vi "Update.vi"(9 "log line":string, 10 "file ref":refnum<file>, 11 "size trigger in":refnum<class "RolloverTrigger.Size.lvclass">) -> (3 "size trigger out":refnum<class "RolloverTrigger.Size.lvclass">)   [LabVIEW 2018, in "GLog.lvlib" / "RolloverTrigger.Size.lvclass"]
doc: "Updates the current file size without touching the filesystem."
uses:
  RolloverTrigger.Size.lvclass
  RolloverTrigger.Size.lvclass/RolloverTrigger.Size.ctl
  d0e10f38-aaa8-410d-b386-210e52cdc805.vi
panel:
  # "Connector Pane"
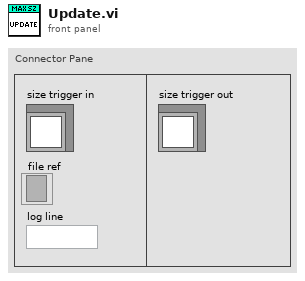
[diagram p1: front panel]
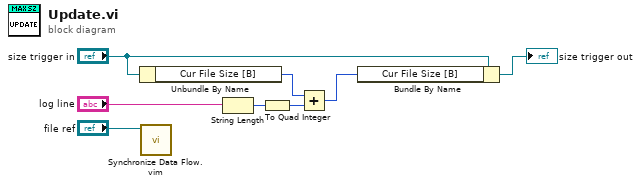
[diagram p0: block diagram]
diagram:
  n1 = Unbundle By Name("size trigger in") -> ("Cur File Size [B]"=w5:i64)
  n2 = call "Synchronize Data Flow.vim"("input 1"="file ref") -> ()  [unwired: 3 in, 4 out]
  n3 = String Length(string="log line") -> (length=w4:i32)
  n4 = To Quad Integer(1:w4) -> (0:w7:i64)
  n5 = Add(x=w5, y=w7) -> (x+y=w2:i64)
  n6 = Bundle By Name(cluster="size trigger in", "Cur File Size [B]"=w2) -> (→"size trigger out":refnum<class "RolloverTrigger.Size.lvclass">)
